vi "WriteRegister.vi"(6 "error in":errorcluster, 7 "string in":string, 8 "value in":i32, 9 "connection ID in":refnum<k5>) -> (0 "error out":errorcluster, 3 "connection ID out":refnum<k5>)   [LabVIEW 2014]
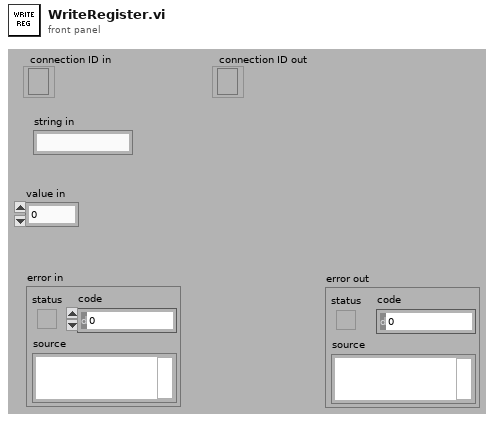
[diagram p1: front panel]
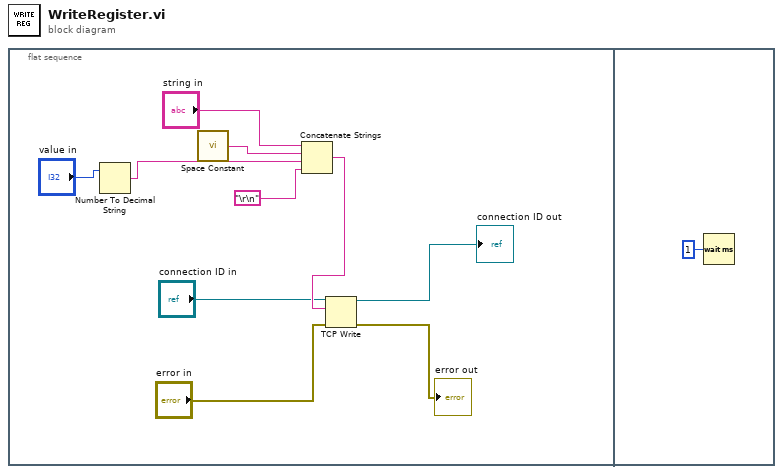
[diagram p0: block diagram]
diagram:
  n1 = flat-sequence {
    frame #0 {
      n2 = Number To Decimal String(number="value in") -> (decimal integer string=w3:string)  [unwired: 1 in]
      n3 = call <vilib>:"Space Constant.vi"() -> ("String"=w1:string)
      n4 = Concatenate Strings("string in", w1, w3, "\r\n") -> (w10:string)
      n5 = TCP Write(connection ID="connection ID in", data in=w10, error in (no error)="error in") -> (connection ID out=→"connection ID out":refnum<k5>, error out=→"error out":errorcluster)  [unwired: 1 in, 1 out]
    }
    frame #1 {
      n6 = Wait (ms)(milliseconds to wait=u32 1) -> ()  [unwired: 1 out]
    }
  }
